vi "File Name of Python Adapter--constant.vi"() -> (3 "File Name of Python Adapter":string)   [LabVIEW 2026]
doc: "This constant defines the name of the productively used python adapter in the generated project."
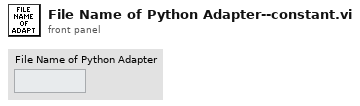
[diagram p1: front panel]
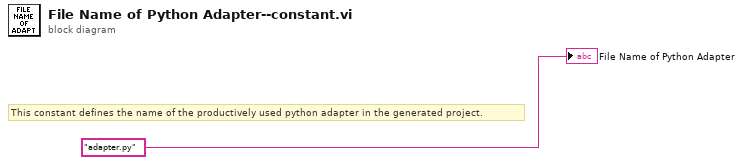
[diagram p0: block diagram]
diagram:
  # "This constant defines the name of the productively used python adapter in the generated project."
  "File Name of Python Adapter" <- "adapter.py" ("File Name of Python Module")
